vi "Configuration Tool Main.vi"() -> ()   [LabVIEW 2015, in "Configuration Tool.lvlib"]
doc: "This is the main VI for the configuration editor."
uses:
  Configuration Tool.lvlib
  Controls/StateCluster.ctl
  <vilib>/NI/Configuration Framework/Repository/NISE_CEF_Repository.lvclass
  <vilib>/NI/Configuration Framework/Node/NodeRef.ctl
  <vilib>/NI/Configuration Framework/Node/NISE_CEF_Node.lvclass
  <vilib>/NI/Configuration Framework/Node/StandardEvents.ctl
  <vilib>/NI/Configuration Framework/Node/UserEventRef.ctl
  <vilib>/NI/Configuration Framework/Controls/EventCluster.ctl
  <vilib>/NI/Configuration Framework/Node/NodeChangeEvent.ctl
  <vilib>/NI/Configuration Framework/Node/CacheState.ctl
  <vilib>/NI/Configuration Framework/Node/RefreshUIEvent.ctl
  <vilib>/NI/Configuration Framework/Node/StopEvent.ctl
  <vilib>/NI/Configuration Framework/glyph manager/glyph manager.ctl
  <vilib>/picture/picture.llb/imagedata.ctl
  Controls/AddMessage.ctl
  Controls/MoveMessage.ctl
  <vilib>/Utility/error.llb/DialogType.ctl
  Classes/CustomDeviceRepo/CustomDeviceRepo.lvclass
  <vilib>/Utility/sysdir.llb/System Directory Type.ctl
  <vilib>/NI/AMC/Read Termination Message.vi
  <vilib>/NI/AMC/Create Single Message.vi
  <vilib>/NI/AMC/Update Message Routing Info.vi
  subVI/Global Settings.vi
  <vilib>/NI/AMC/Globals.vi
  <vilib>/NI/AMC/Send Message.vi
  <vilib>/NI/AMC/AMC.lvlib
  <vilib>/NI/Configuration Framework/NISE_CEF_TreeControl.lvlib
  <vilib>/NI/Configuration Framework/glyph manager/glyph manager.lvlib
panel:
  in  "Target Project":string(combo)
  in  "VeriStand Version":enum16{"2013", "2014", "2015", "2016"}(ring)=enum."2015"
  in  "View":string(tree)
  in  "Exit":bool
  out "Status":string
  # "Custom Device XML Editor"
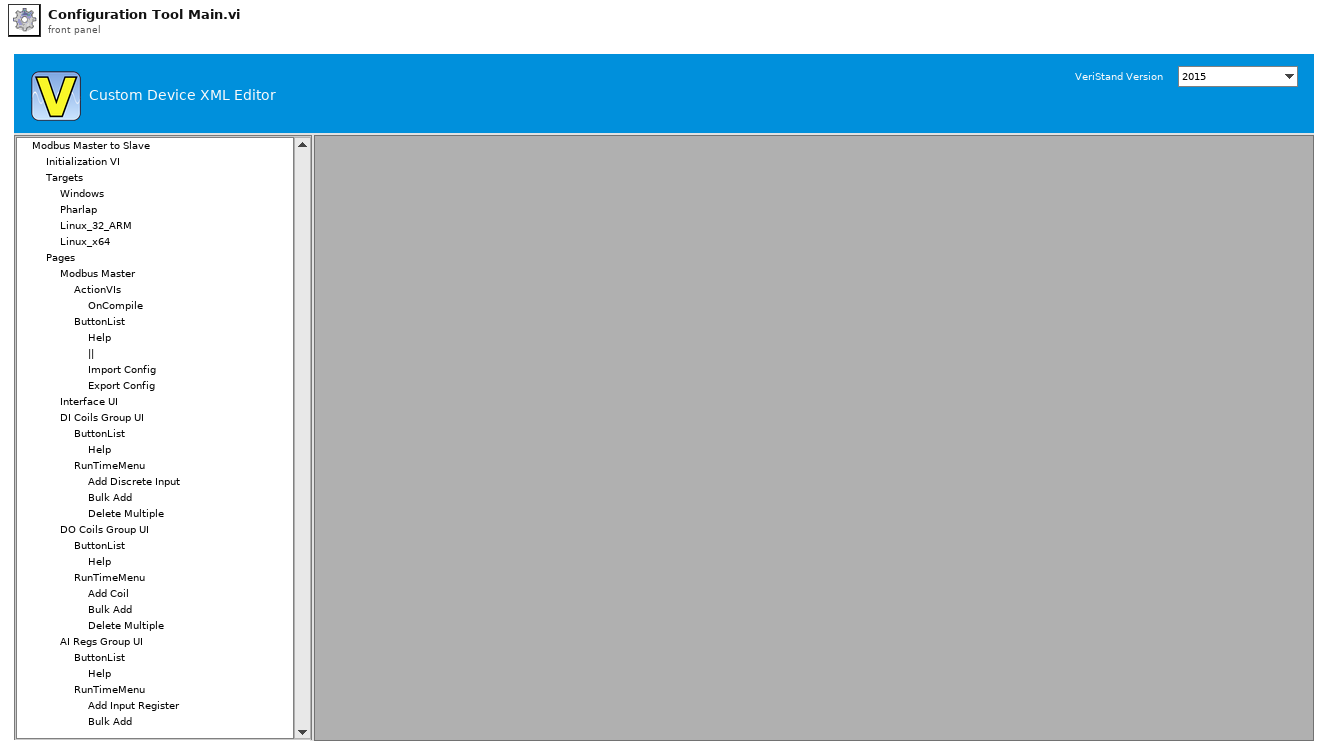
[diagram p1: front panel]
types:
  T1 = typedef "Configuration Tool.lvlib/StateCluster.ctl" = cluster{"repository":refnum<class "NISE_CEF_Repository.lvclass">, "root":T2, "unsaved changes":bool, "current path":path, "standard events":T3, "classes path":path, "glyph manager":T9}
  T2 = typedef "NISE_CEF_Node.lvclass/NodeRef.ctl" = refnum<data-value>
  T3 = typedef "NISE_CEF_Node.lvclass/StandardEvents.ctl" = cluster{"user event":T4, "node change":T5, "cache state":T6, "refresh UI":T7, "stop event":T8}
  T4 = typedef "NISE_CEF_Node.lvclass/UserEventRef.ctl" = refnum<user-event>
  T5 = typedef "NISE_CEF_Node.lvclass/NodeChangeEvent.ctl" = refnum<user-event>
  T6 = typedef "NISE_CEF_Node.lvclass/CacheState.ctl" = refnum<user-event>
  T7 = typedef "NISE_CEF_Node.lvclass/RefreshUIEvent.ctl" = refnum<user-event>
  T8 = typedef "NISE_CEF_Node.lvclass/StopEvent.ctl" = refnum<user-event>
  T9 = typedef "glyph manager.lvlib/glyph manager.ctl" = cluster{"search paths":path[], "glyph map":variant, "base glyphs":T10[], "desired overlays":string[]}
  T10 = typedef "imagedata.ctl" = cluster{"image type":i32, "image depth":i32, "image":u8[], "mask":u8[], "colors":u32[], "Rectangle":cluster{"left":i16, "top":i16, "right":i16, "bottom":i16}}
  T11 = cluster{"Names":string[], "Project refs":refnum<vi>[]}
  T12 = typedef "AMC.lvlib/Message Queue.ctl" = refnum<queue>
  T13 = typedef "Configuration Tool.lvlib/AddMessage.ctl" = cluster{"node type":string, "to add to":string}
  T14 = typedef "Configuration Tool.lvlib/MoveMessage.ctl" = cluster{"node ref":T2, "new parent":T2}
  T15 = typedef "Configuration Tool.lvlib/FilePaths.ctl" = cluster{"glyphs":path, "classes":path}
  T16 = typedef "DialogType.ctl" = u16
  T17 = typedef "System Directory Type.ctl" = i32
  T18 = typedef "NISE_CEF_Node.lvclass/Summary.ctl" = cluster{"ID":string, "parent ID":string, "node type":string, "text":string, "additional text":string, "glyph":string, "depth":i32, "glyph overlay":string}
  T19 = typedef "LVPoint32TypeDef.ctl" = cluster{"Horizontal":i32, "Vertical":i32}
  T20 = cluster{"data name":string, "drag data":variant}[]
  T21 = typedef "NISE_CEF_Node.lvclass/NodeMenuOptions.ctl" = cluster{"removable":bool, "movable":bool, "duplicate":bool}
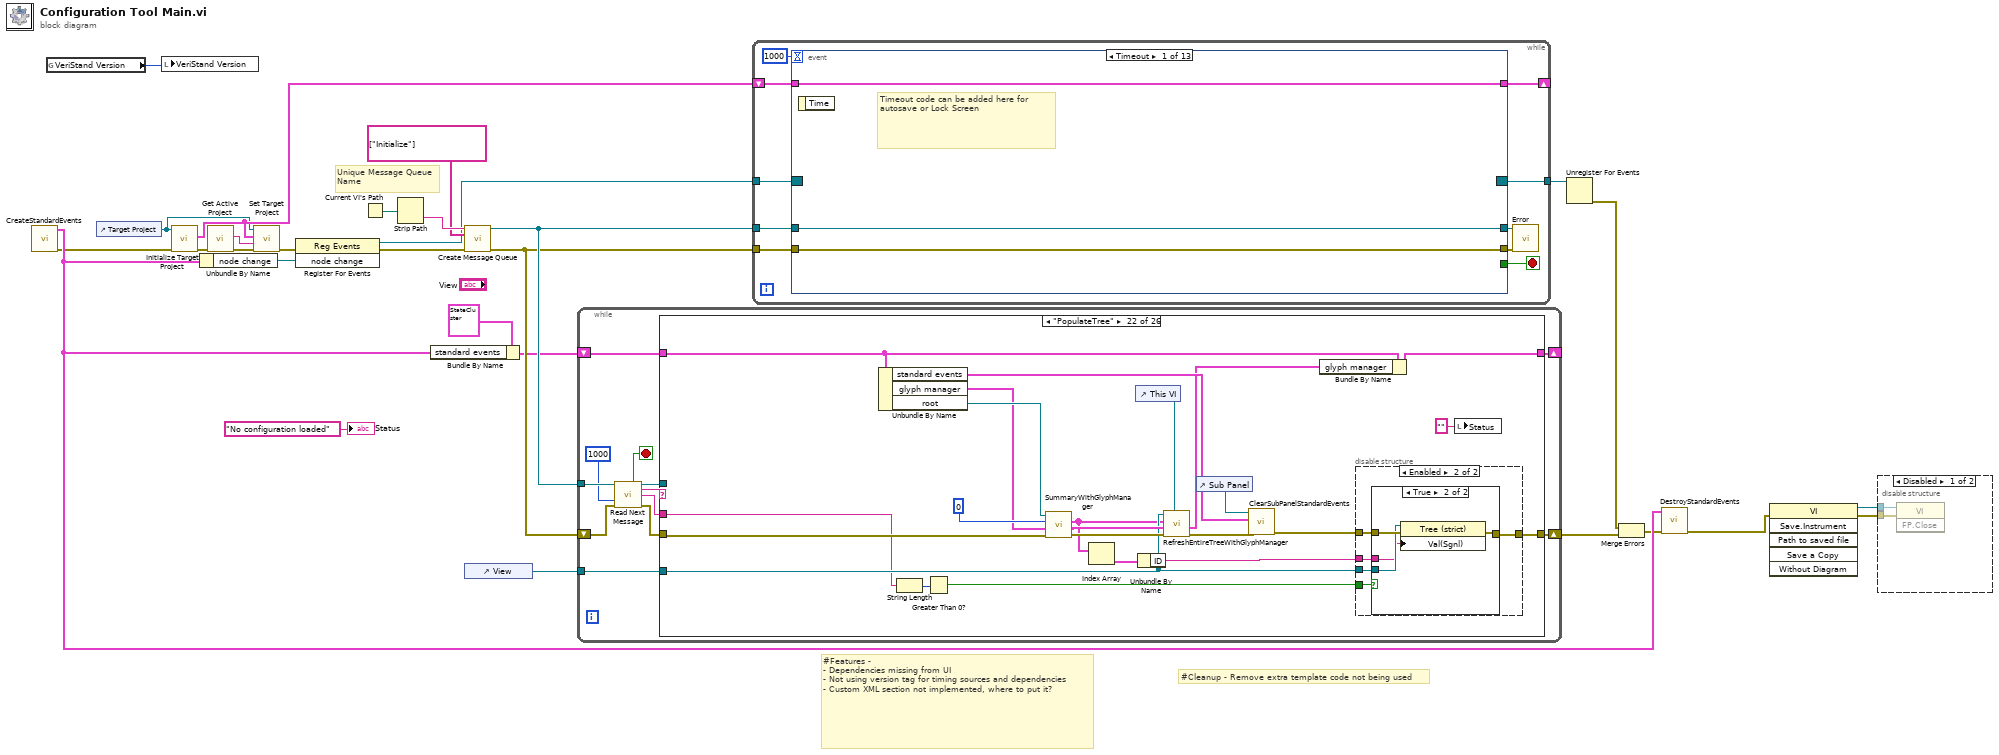
[diagram p0: block diagram]
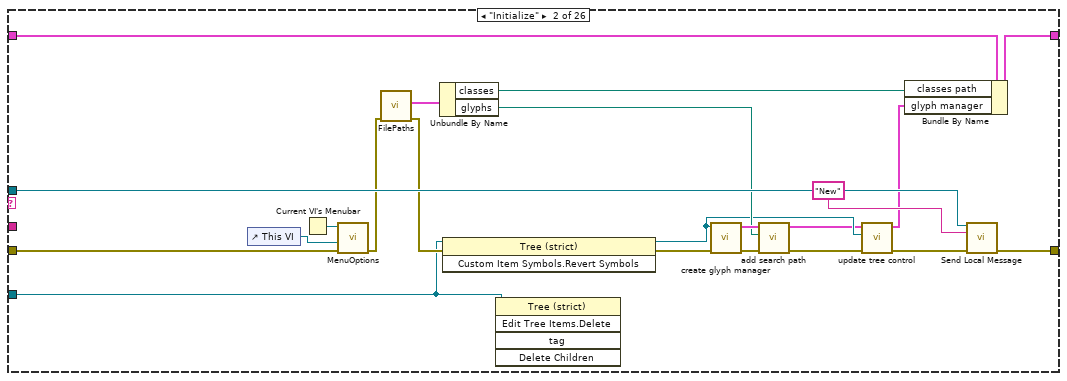
[diagram p4: hidden frame]
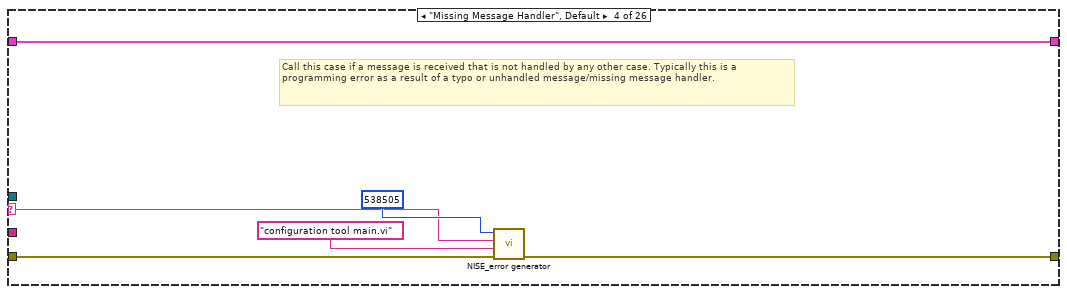
[diagram p6: hidden frame]
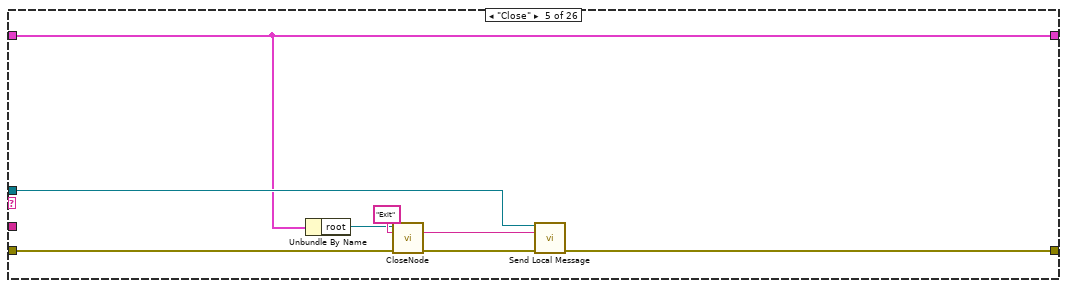
[diagram p7: hidden frame]
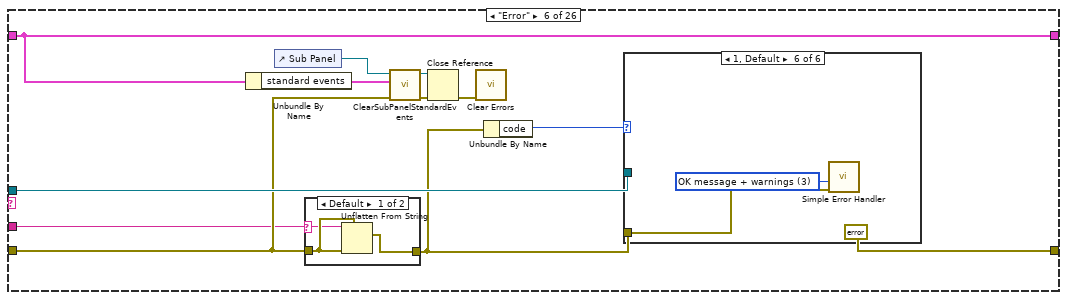
[diagram p8: hidden frame]
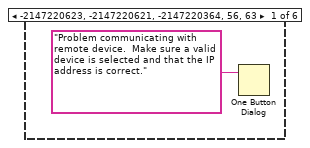
[diagram p10: hidden frame]
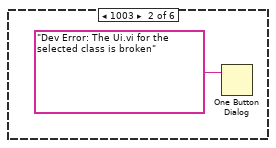
[diagram p11: hidden frame]
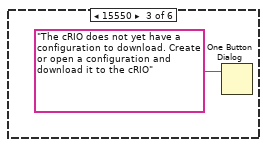
[diagram p12: hidden frame]
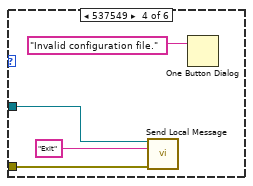
[diagram p13: hidden frame]
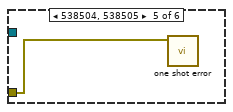
[diagram p14: hidden frame]
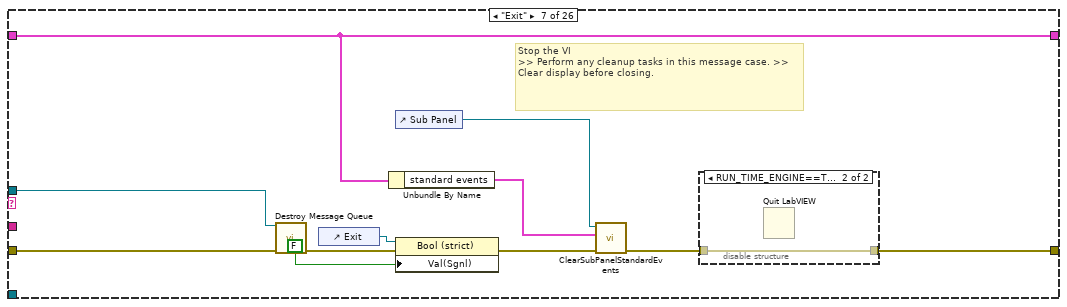
[diagram p15: hidden frame]
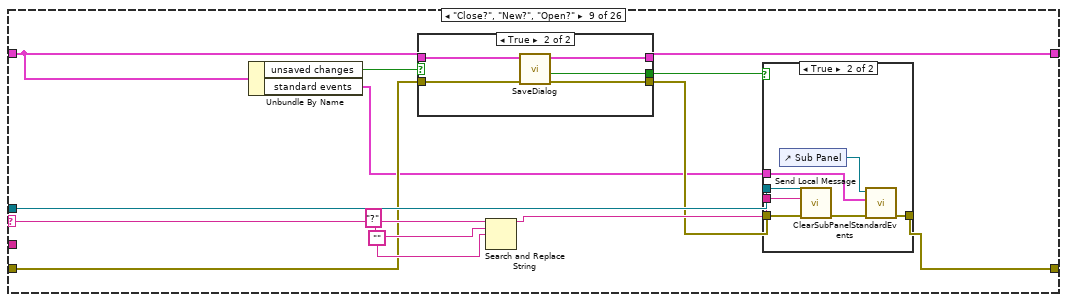
[diagram p18: hidden frame]
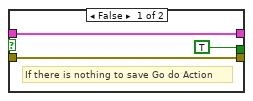
[diagram p19: hidden frame]
diagram:
  # "#Cleanup - Remove extra template code not being used"
  # "#Features - \n- Dependencies missing from UI\n- Not using version tag for timing sources and dependencies\n- Custom XML section not implemented, where to put it?"
  # "Unique Message Queue Name"
  n1 = call <vilib>:"CreateStandardEvents.vi"() -> ("error out"=w6:errorcluster, "standard events"=w18:T3)  [unwired: 10 in]
  n2 = global read "Global Settings.vi" "VeriStand Version"() -> (w12:enum16{"2013", "2014", "2015", "2016"})
  n3 = control-ref of="Target Project"() -> (w7:refnum<vi>)
  n4 = local write "VeriStand Version"(w12) -> ()
  n5 = call "Initialize Target Project.vi"("error in (no error)"=w6, "ComboBox in"=w7) -> ("error out"=w11:errorcluster, "Projects"=w9:T11)  [unwired: 8 in]
  n6 = Unbundle By Name(w18) -> ("node change"=w23:T5)
  n7 = call "Get Active Project.vi"("error in (no error)"=w11) -> ("error out"=w10:errorcluster, "Name"=w8:string)  [unwired: 7 in, 2 out]
  n8 = call "Set Target Project.vi"("error in (no error)"=w10, "Target Project"=w8, "Projects"=w9, "ComboBox Ref"=w7) -> ("error out"=w5:errorcluster)  [unwired: 7 in]
  n9 = register-events(error in=w5, w23) -> (reference out=w17:refnum<event-registration>, error out=w22:errorcluster)  [unwired: 1 in]
  n10 = Current VI's Path() -> (path=w27:path)
  n11 = Strip Path(path=w27) -> (name=w28:string)  [unwired: 1 out]
  n12 = Bundle By Name(cluster=T1 {"repository"=refnum, "root"=refnum, "unsaved changes"=FALSE, "current path"=path "", "standard events"={"user event"=refnum, "node change"=refnum, "cache state"=refnum, "refresh UI"=refnum, "stop event"=refnum}, "classes path"=path "", "glyph manager"={"search paths"=[], "glyph map"=variant, "base glyphs"=[], "desired overlays"=[]}}, "standard events"=w18) -> (w20:T1)
  n13 = call <vilib>:"Create Message Queue.vi"("message queue name"=w28, "initial message names"=string[] ["Initialize"], "error in"=w22) -> ("message queue out"=w25:T12, "error out"=w24:errorcluster)  [unwired: 11 in]
  n14 = control-ref of="View"() -> (w16:refnum<vi>)
  n15 = while "Message Processor" {
    shift-right: [w36] -> w19
    shift-left: w24 -> [w35]
    tunnel: w25 -> [w34]
    shift-right: [w32] -> _
    shift-left: w20 -> [w31]
    tunnel: w16 -> [w29]
    stop <- w40 stop-if-true
    n16 = call <vilib>:"Read Next Message.vi"("message queue in"=w34, "timeout (1 ms)"=1000, "error in"=w35) -> ("exit process?"=w40:bool, "message queue out"=w30:T12, "message name"=w39:string, "message value"=w38:string, "error out"=w37:errorcluster)  [unwired: 5 in, 3 out]
    n17 = case shown="\"PopulateTree\"" w39 {
      selector: w39 -> [_ _ _ w68 _ _ _ _ w129 _ _ _ _ _ _ _ _ _ w385 _ _ _ _ _ _ _]
      tunnel: w38 -> [_ _ _ _ _ w81 _ _ _ _ _ _ _ _ w294 _ w346 w363 w383 w435 w459 w471 _ w520 w540 w547]
      tunnel: w37 -> [w42 w64 w66 w71 w74 w84 w116 w120 w122 w160 w180 w220 w264 w286 w301 w314 w339 w362 w388 w437 w458 w488 w510 w519 w538 w548]
      tunnel: [w42 w60 w66 w69 w78 errorcluster {"status"=FALSE, "code"=0, "source"=""} ("error out") w108 w120 w133 w166 w176 w225 w261 w288 w298 w314 w318 w366 w391 w439 w455 w475 w506 w516 w533 w546] -> w36
      tunnel: [w41 w56 w65 w72 w76 w88 w107 w119 w124 w164 w181 w228 w267 w287 w295 w313 w334 w359 w392 w438 w460 w481 w509 w514 w541 w543] -> w32
      tunnel: w31 -> [w41 w57 w65 w72 w76 w88 w107 w119 w125 w162 w182 w229 w266 w285 w296 w313 w337 w360 w392 w430 w460 w490 w509 w514 w541 w549]
      tunnel: w30 -> [_ w59 _ _ w77 w91 w115 _ w132 w165 w178 w227 _ _ w297 _ w315 _ w386 _ _ _ _ w515 w532 w545]
      tunnel: w29 -> [_ w43 _ _ _ _ _ _ _ _ _ _ _ _ _ _ w335 w355 w380 w432 w453 w477 _ _ _ _]
      frame "------------Generic Operations------------" {
        # "Dummy case to add a seperation in the Case Structure menu"
      }
      frame "Initialize" {
        n18 = control-ref of="This VI"() -> (w63:refnum<vi>)
        n19 = Current VI's Menubar() -> (w62:refnum<k9>)
        n20 = call "MenuOptions.vi"("error in"=w64, "VI ref"=w63, "menu ref in"=w62) -> ("error out"=w55:errorcluster)  [unwired: 7 in, 1 out]
        n21 = call "FilePaths.vi"("error in"=w55) -> ("error out"=w48:errorcluster, "paths"=w58:T15)  [unwired: 9 in]
        n22 = Unbundle By Name(w58) -> ("classes"=w54:path, "glyphs"=w50:path)
        n23 = invoke class="Tree (strict)" method="Custom Item Symbols.Revert Symbols"(reference=w43, error in=w48) -> (reference out=w46:refnum<vi>, error out=w47:errorcluster)  [unwired: 1 in, 1 out]
        n24 = invoke class="Tree (strict)" method="Edit Tree Items.Delete"(reference=w43) -> ()  [unwired: 4 in, 5 out]
        n25 = call <vilib>:"create glyph manager.vi"("error in"=w47, "tree ref (for default symbols)"=w46) -> ("error out"=w53:errorcluster, "glyph manager"=w52:T9)  [unwired: 8 in]
        n26 = call <vilib>:"add search path.vi"("error in"=w53, "search path"=w50, "glyph manager in"=w52) -> ("error out"=w45:errorcluster, "glyph manager out"=w44:T9)  [unwired: 7 in]
        n27 = call <vilib>:"update tree control.vi"("error in"=w45, "tree reference"=w46, "glyph manager in"=w44) -> ("error out"=w51:errorcluster, "glyph manager out"=w49:T9)  [unwired: 7 in]
        n28 = Bundle By Name(cluster=w57, "classes path"=w54, "glyph manager"=w49) -> (w56:T1)
        n29 = call <vilib>:"Send Local Message.vi"("message queue in"=w59, "message name"="New" ("Message Name"), "error in"=w51) -> ("error out"=w60:errorcluster)  [unwired: 10 in, 2 out]
      }
      frame "", "Idle" {
      }
      frame "Missing Message Handler", Default {
        # "Call this case if a message is received that is not handled by any other case. Typically this is a programming error as a result of a typo or unhandled message/missing message handler."
        n30 = call <vilib>:"NISE_error generator.vi"("error in"=w71, "source"="configuration tool main.vi", "append error message"=w68, "error code (0)"=538505) -> ("error out"=w69:errorcluster)  [unwired: 5 in]
      }
      frame "Close" {
        n31 = Unbundle By Name(w76) -> ("root"=w75:T2)
        n32 = call <vilib>:"CloseNode.vi"("error in"=w74, "node ref"=w75) -> ("error out"=w73:errorcluster)  [unwired: 9 in]
        n33 = call <vilib>:"Send Local Message.vi"("message queue in"=w77, "message name"="Exit", "error in"=w73) -> ("error out"=w78:errorcluster)  [unwired: 10 in, 2 out]
      }
      frame "Error" {
        n34 = Unbundle By Name(w88) -> ("standard events"=w80:T3)
        n35 = control-ref of="Sub Panel"() -> (w87:refnum<vi>)
        n36 = case shown="Default" w81 {
          selector: w81 -> [w93 _]
          tunnel: w84 -> [w94 w95]
          tunnel: [w92 w95] -> w83
          frame Default {
            n37 = Unflatten From String(type=w94, binary string=w93, error in (no error)=w94) -> (value=w92:errorcluster)  [unwired: 2 in, 2 out]
          }
          frame "" {
          }
        }
        n38 = call <vilib>:"ClearSubPanelStandardEvents.vi"("error in"=w84, "standard events"=w80, "sub panel ref in"=w87) -> ("error out"=w86:errorcluster, "sub panel ref out"=w85:refnum<vi>)  [unwired: 7 in]
        n39 = Close Reference(reference=w85, error in (no error)=w86) -> (error out=w82:errorcluster)
        n40 = call <vilib>:"Clear Errors.vi"("error in (no error)"=w82) -> ()  [unwired: 5 in, 2 out]
        n41 = Unbundle By Name(w83) -> ("code"=w89:i32)
        n42 = case shown="1, Default" w89 {
          tunnel: w91 -> [_ _ _ w101 _ _]
          tunnel: w83 -> [_ _ _ w100 w103 w105]
          frame -2147220623, -2147220621, -2147220364, 56, 63 {
            n43 = One Button Dialog(message="Problem communicating with remote device.  Make sure a valid device is selected and that the IP address is correct.") -> ()  [unwired: 1 in, 1 out]
          }
          frame 1003 {
            n44 = One Button Dialog(message="Dev Error: The Ui.vi for the selected class is broken") -> ()  [unwired: 1 in, 1 out]
          }
          frame 15550 {
            n45 = One Button Dialog(message="The cRIO does not yet have a configuration to download. Create or open a configuration and download it to the cRIO") -> ()  [unwired: 1 in, 1 out]
          }
          frame 537549 {
            n46 = call <vilib>:"Send Local Message.vi"("message queue in"=w101, "message name"="Exit", "error in"=w100) -> ()  [unwired: 10 in, 3 out]
            n47 = One Button Dialog(message="Invalid configuration file.") -> ()  [unwired: 1 in, 1 out]
          }
          frame 538504, 538505 {
            n48 = call <vilib>:"one shot error.vi"("error in"=w103) -> ()  [unwired: 11 in]
          }
          frame 1, Default {
            w104 = T16 3 items=["no dialog", "OK message", "continue or stop message", "OK message + warnings", "continue/stop + warnings"] ("type of dialog (OK msg:1)")
            n49 = call <vilib>:"Simple Error Handler.vi"("type of dialog (OK msg:1)"=w104, "error in (no error)"=w105) -> ()  [unwired: 8 out]
          }
        }
      }
      frame "Exit" {
        # "Stop the VI                                                                             >> Perform any cleanup tasks in this message case. >> Clear display before closing."
        n50 = call <vilib>:"Destroy Message Queue.vi"("message queue in"=w115, "error in"=w116) -> ("error out"=w112:errorcluster)  [unwired: 11 in, 2 out]
        n51 = control-ref of="Exit"() -> (w114:refnum<vi>)
        n52 = Unbundle By Name(w107) -> ("standard events"=w106:T3)
        n53 = control-ref of="Sub Panel"() -> (w111:refnum<vi>)
        n54 = property class="Bool (strict)"(reference=w114, error in=w112, "Val(Sgnl)"=FALSE ("Exit")) -> (error out=w110:errorcluster)  [unwired: 1 out]
        n55 = call <vilib>:"ClearSubPanelStandardEvents.vi"("error in"=w110, "standard events"=w106, "sub panel ref in"=w111) -> ("error out"=w109:errorcluster)  [unwired: 7 in, 1 out]
        n56 = disable-structure shown="RUN_TIME_ENGINE==True" {
          disable-tunnel: [w117 w118] -> w108
          disable-tunnel: w109 -> [w117 w118]
          frame condition #0 (active) {
          }
          frame condition #1 {
            n57 = Quit LabVIEW() -> ()  [unwired: 1 in]
          }
        }
      }
      frame "------------Menu Operations--------------" {
        # "Dummy case to add a seperation in the Case Structure menu"
      }
      frame "Close?", "New?", "Open?" {
        n58 = Unbundle By Name(w125) -> ("unsaved changes"=w127:bool, "standard events"=w121:T3)
        n59 = case shown="True" w127 {
          tunnel: [TRUE ("SaveFlag") w141] -> w126
          tunnel: w125 -> [w135 w140]
          tunnel: [w135 w139] -> w124
          tunnel: w122 -> [w134 w138]
          tunnel: [w134 w137] -> w123
          frame False {
            # "If there is nothing to save Go do Action"
          }
          frame True {
            n60 = call "SaveDialog.vi"("error in"=w138, "state in"=w140) -> ("error out"=w137:errorcluster, "new"=w141:bool, "state out"=w139:T1)  [unwired: 7 in]
          }
        }
        n61 = Search and Replace String(input string=w129, search string="?", replace string="") -> (result string=w128:string)  [unwired: 5 in, 3 out]
        n62 = case shown="True" w126 {
          tunnel: w123 -> [w142 w149]
          tunnel: [w142 w145] -> w133
          tunnel: w132 -> [_ w148]
          tunnel: w128 -> [_ w147]
          tunnel: w121 -> [_ w143]
          frame False {
          }
          frame True {
            n63 = control-ref of="Sub Panel"() -> (w144:refnum<vi>)
            n64 = call <vilib>:"Send Local Message.vi"("message queue in"=w148, "message name"=w147, "error in"=w149) -> ("error out"=w146:errorcluster)  [unwired: 10 in, 2 out]
            n65 = call <vilib>:"ClearSubPanelStandardEvents.vi"("error in"=w146, "standard events"=w143, "sub panel ref in"=w144) -> ("error out"=w145:errorcluster)  [unwired: 7 in, 1 out]
          }
        }
      }
      frame "New" {
        # "#Change - Won't allow creating so changing unsaved constant to F"
        n66 = Unbundle By Name(w162) -> ("classes path"=w161:path)
        n67 = Current VI's Menubar() -> (w156:refnum<k9>)
        n68 = call-dynamic "Initialize.vi"("error in"=w160, "path"=w161, "repository in"=refnum<class "CustomDeviceRepo.lvclass"> refnum ("CustomDeviceRepo.lvclass")) -> ("error out"=w159:errorcluster, "repository out"=w158:refnum<class "CustomDeviceRepo.lvclass">)  [unwired: 7 in]
        n69 = call-dynamic "GenerateMenu.vi"("error in"=w159, "menu ref in"=w156, "NISE_CEF_Repository in"=w158) -> ("error out"=w155:errorcluster, "NISE_CEF_Repository out"=w157:refnum<class "CustomDeviceRepo.lvclass">)  [unwired: 6 in, 1 out]
        n70 = call "Get Active Project.vi"() -> ("No Active Project?"=w153:bool)  [unwired: 8 in, 3 out]
        n71 = Bundle By Name(cluster=w162, "unsaved changes"=FALSE ("SaveFlag"), "repository"=w157) -> (w164:T1)
        n72 = Select(t="Idle", s=w153, f="Open Active") -> (s? t:f=w150:string)
        n73 = call <vilib>:"Send Local Message.vi"("message queue in"=w165, "message name"=w150, "error in"=w155) -> ("error out"=w166:errorcluster)  [unwired: 10 in, 2 out]
      }
      frame "Open" {
        w175 = T17 6 items=["User Home"=0, "User Desktop"=1, "User Documents"=2, "User Application Data"=3, "User Preferences"=4, "User Temporary"=5, "Public Documents"=6, "Public Application Data"=7, "Public Preferences"=8, "Public Cache"=13, "System Core Libraries"=9, "System Installed Libraries"=10, "Application Files"=11, "Boot Volume Root"=12] ("system directory type")
        n74 = global read "Global Settings.vi" "VeriStand Version"() -> (w168:enum16{"2013", "2014", "2015", "2016"})
        n75 = Format Into String(w168) -> (resulting string=w167:string)  [unwired: 3 in, 1 out]
        n76 = Search and Replace String(input string="National Instruments\\NI VeriStand XXXX\\Custom Devices", search string="XXXX", replace string=w167) -> (result string=w171:string)  [unwired: 5 in, 3 out]
        n77 = call <vilib>:"Get System Directory.vi"("system directory type"=w175) -> ("system directory"=w172:path)  [unwired: 10 in]
        n78 = Build Path(base path=w172, name or relative path=w171) -> (appended path=w170:path)
        n79 = in-place {
          in-place-border: w180 -> [w188]
          in-place-border: [w187] -> w177
          in-place-border: w170 -> [w183]
          n80 = in-place-cluster #1(w182) -> ("current path"=w185:path, "repository"=w196:refnum<class "NISE_CEF_Repository.lvclass">, "root"=w192:T2)  [unwired: 1 out]
          n81 = call "FileDialog.vi"("error in"=w188, "start path"=w183) -> ("error out"=w189:errorcluster, "cancelled"=w190:bool, "selected path"=w186:path)  [unwired: 7 in]
          n82 = Compound Arithmetic op=OR(invert w190) -> (w191:bool)
          n83 = case shown="True" w191 {
            tunnel: w196 -> [w197 w209]
            tunnel: [w197 w207] -> w194
            tunnel: [w198 w205] -> w187
            tunnel: [w199 w204] -> w193
            tunnel: w186 -> [_ w202]
            tunnel: w189 -> [w198 w201]
            tunnel: w192 -> [w199 w200]
            frame False {
            }
            frame True {
              n84 = call-dynamic "Open.vi"("error in"=w201, "file path"=w202, "repository in"=w209) -> ("error out"=w206:errorcluster, "invalid?"=w203:bool, "repository out"=w208:refnum<class "NISE_CEF_Repository.lvclass">)  [unwired: 6 in]
              n85 = case shown="False" w203 {
                tunnel: w208 -> [w214 w217]
                tunnel: [w213 w217] -> w207
                tunnel: w206 -> [w212 w216]
                tunnel: [w211 w216] -> w205
                tunnel: [w210 w215] -> w204
                tunnel: w200 -> [_ w215]
                frame False {
                  n86 = call-dynamic "WriteTree.vi"("error in"=w212, "repository in"=w214) -> ("error out"=w211:errorcluster, "root"=w210:T2, "repository out"=w213:refnum<class "NISE_CEF_Repository.lvclass">)  [unwired: 7 in]
                }
                frame True {
                }
              }
            }
          }
          n87 = Select(t=w185, s=w187, f=w186) -> (s? t:f=w184:path)
          n88 = in-place-cluster #1("current path"=w184, "unsaved changes"=FALSE ("SaveFlag"), "repository"=w194, "root"=w193) -> (w181:T1)
        }
        n89 = call <vilib>:"Send Local Message.vi"("message queue in"=w178, "message name"="PopulateTree", "message value"="Zero", "error in"=w177) -> ("error out"=w176:errorcluster)  [unwired: 9 in, 2 out]
      }
      frame "Open Active" {
        n90 = global read "Global Settings.vi" "Target Project Ref"() -> (w223:refnum<vi>)
        n91 = call "Search Project for XML Files.vi"("error in (no error)"=w220, "project reference"=w223) -> ("error out"=w219:errorcluster, "xml files found"=w222:path[])  [unwired: 8 in]
        n92 = Empty Array?(array=w222) -> (empty?=w221:bool)
        n93 = case shown="True" w221 {
          tunnel: w229 -> [w236 w260]
          tunnel: [w235 w260] -> w228
          tunnel: w219 -> [w234 w259]
          tunnel: [w233 w259] -> w226
          tunnel: w222 -> [w231 _]
          tunnel: ["PopulateTree" "Idle"] -> w218
          frame False {
            n94 = Index Array(array=w231) -> (element=w232:path)  [unwired: 1 in]
            n95 = in-place {
              in-place-border: w234 -> [w244]
              in-place-border: [w243] -> w233
              in-place-border: w232 -> [w237]
              n96 = in-place-cluster #2(w236) -> ("current path"=w242:path, "repository"=w249:refnum<class "NISE_CEF_Repository.lvclass">, "root"=w245:T2)  [unwired: 1 out]
              n97 = call-dynamic "Open.vi"("error in"=w244, "file path"=w237, "repository in"=w249) -> ("error out"=w239:errorcluster, "invalid?"=w238:bool, "repository out"=w240:refnum<class "NISE_CEF_Repository.lvclass">)  [unwired: 6 in]
              n98 = case shown="False" w238 {
                tunnel: w240 -> [w254 w257]
                tunnel: [w253 w257] -> w247
                tunnel: w239 -> [w252 w256]
                tunnel: [w251 w256] -> w243
                tunnel: [w250 w255] -> w246
                tunnel: w245 -> [_ w255]
                frame False {
                  n99 = call-dynamic "WriteTree.vi"("error in"=w252, "repository in"=w254) -> ("error out"=w251:errorcluster, "root"=w250:T2, "repository out"=w253:refnum<class "NISE_CEF_Repository.lvclass">)  [unwired: 7 in]
                }
                frame True {
                }
              }
              n100 = Select(t=w242, s=w243, f=w237) -> (s? t:f=w241:path)
              n101 = in-place-cluster #2("current path"=w241, "unsaved changes"=FALSE ("SaveFlag"), "repository"=w247, "root"=w246) -> (w235:T1)
            }
          }
          frame True {
          }
        }
        n102 = call <vilib>:"Send Local Message.vi"("message queue in"=w227, "message name"=w218, "message value"="Zero", "error in"=w226) -> ("error out"=w225:errorcluster)  [unwired: 9 in, 2 out]
      }
      frame "Save" {
        n103 = in-place {
          in-place-border: w264 -> [w271]
          in-place-border: [w270] -> w263
          in-place-border: [w268] -> w262
          n104 = in-place-cluster #3(w266) -> ("current path"=w269:path, "root"=w272:T2, "repository"=w274:refnum<class "NISE_CEF_Repository.lvclass">)
          n105 = Empty String/Path?(string/path=w269) -> (empty?=w268:bool)
          n106 = call-dynamic "ReadTree.vi"("error in"=w271, "root"=w272, "repository in"=w274) -> ("error out"=w270:errorcluster, "repository out"=w273:refnum<class "NISE_CEF_Repository.lvclass">)  [unwired: 7 in]
          n107 = in-place-cluster #3("current path"=w269, "root"=w272, "repository"=w273) -> (w265:T1)
        }
        n108 = case shown="False" w262 {
          tunnel: w265 -> [w278 w280]
          tunnel: [w277 w279] -> w267
          tunnel: [w276 w281] -> w261
          tunnel: w263 -> [w275 w282]
          frame False {
            n109 = call "Save.vi"("error in"=w275, "state in"=w278) -> ("error out"=w276:errorcluster, "state out"=w277:T1)  [unwired: 8 in]
          }
          frame True {
            # "Empty path use Dialog"
            n110 = call "SaveAs.vi"("error in"=w282, "state in"=w280) -> ("error out"=w281:errorcluster, "state out"=w279:T1)  [unwired: 7 in, 1 out]
          }
        }
      }
      frame "SaveAs" {
        n111 = in-place {
          in-place-border: w286 -> [w290]
          in-place-border: [w289] -> w284
          n112 = in-place-cluster #4(w285) -> ("root"=w291:T2, "repository"=w293:refnum<class "NISE_CEF_Repository.lvclass">)
          n113 = call-dynamic "ReadTree.vi"("error in"=w290, "root"=w291, "repository in"=w293) -> ("error out"=w289:errorcluster, "repository out"=w292:refnum<class "NISE_CEF_Repository.lvclass">)  [unwired: 7 in]
          n114 = in-place-cluster #4("root"=w291, "repository"=w292) -> (w283:T1)
        }
        n115 = call "SaveAs.vi"("error in"=w284, "state in"=w283) -> ("error out"=w288:errorcluster, "state out"=w287:T1)  [unwired: 7 in, 1 out]
      }
      frame "Custom View" {
        n116 = in-place {
          in-place-border: w301 -> [w312]
          in-place-border: [w311] -> w299
          in-place-border: w294 -> [w302]
          n117 = in-place-cluster #5(w296) -> ("repository"=w306:refnum<class "NISE_CEF_Repository.lvclass">, "root"=w305:T2)
          n118 = call-dynamic "ReadTree.vi"("error in"=w312, "root"=w305, "repository in"=w306) -> ("error out"=w309:errorcluster, "repository out"=w308:refnum<class "NISE_CEF_Repository.lvclass">)  [unwired: 7 in]
          n119 = call-dynamic "CustomView.vi"("error in"=w309, "view name"=w302, "repository in"=w308) -> ("error out"=w310:errorcluster, "repository out"=w307:refnum<class "NISE_CEF_Repository.lvclass">)  [unwired: 7 in]
          n120 = call-dynamic "WriteTree.vi"("error in"=w310, "repository in"=w307) -> ("error out"=w311:errorcluster, "root"=w303:T2, "repository out"=w304:refnum<class "NISE_CEF_Repository.lvclass">)  [unwired: 7 in]
          n121 = in-place-cluster #5("repository"=w304, "root"=w303) -> (w295:T1)
        }
        n122 = call <vilib>:"Send Local Message.vi"("message queue in"=w297, "message name"="PopulateTree", "error in"=w299) -> ("error out"=w298:errorcluster)  [unwired: 10 in, 2 out]
      }
      frame "-------TreeControl Operations-----------" {
        # "Dummy case to add a seperation in the Case Structure menu"
      }
      frame "AddNode" {
        # "#Change - Added ability for added nodes\nto then add children"
        # "#Change - Had to make own copy\nof add node since CEF framework\ndoesn't let you pass params to init"
        # "#Change - Look for potential\ndashes for menu items with\nparameterized options"
        n123 = Unflatten From String(type=T13 {"node type"="", "to add to"=""} ("input cluster"), binary string=w346) -> (value=w344:T13)  [unwired: 3 in, 2 out]
        n124 = Unbundle By Name(w344) -> ("to add to"=w342:string, "node type"=w324:string)
        n125 = Match Pattern(string=w324, regular expression="\\-") -> (before substring=w323:string, after substring=w322:string)  [unwired: 1 in, 2 out]
        n126 = in-place {
          in-place-border: w339 -> [w352]
          in-place-border: [w351] -> w338
          in-place-border: w323 -> [w350]
          in-place-border: [w349] -> w336
          n127 = in-place-cluster #6(w337) -> ("repository"=w354:refnum<class "NISE_CEF_Repository.lvclass">)
          n128 = call-dynamic "GetClassPath.vi"("error in"=w352, "class name"=w350, "Repository in"=w354) -> ("error out"=w351:errorcluster, "class path"=w349:path, "Repository out"=w353:refnum<class "NISE_CEF_Repository.lvclass">)  [unwired: 6 in]
          n129 = in-place-cluster #6("repository"=w353) -> (w331:T1)
        }
        n130 = Unbundle By Name(w331) -> ("glyph manager"=w330:T9)
        n131 = call <vilib>:"Get LV Class Default Value.vi"("error in (no error)"=w338, "class path"=w336) -> ("error out"=w347:errorcluster, "object"=w348:refnum<class>)  [unwired: 8 in]
        n132 = To More Specific Class(target class=refnum<class "NISE_CEF_Node.lvclass"> refnum ("Node.lvclass"), reference=w348, error in=w347) -> (specific class reference=w332:refnum<class "NISE_CEF_Node.lvclass">, error out=w333:errorcluster)
        n133 = call-dynamic "AddGlyphtoGManager.vi"("error in"=w333, "glyph manager"=w330, "NISE_CEF_Node in"=w332) -> ("error out"=w328:errorcluster, "glyph manager out"=w329:T9, "NISE_CEF_Node out"=w327:refnum<class "NISE_CEF_Node.lvclass">)  [unwired: 6 in]
        n134 = Match Pattern(string=w322, regular expression="\\-") -> (before substring=w320:string, after substring=w317:string)  [unwired: 1 in, 2 out]
        n135 = call "Modified Framework AddNode.vi"("parameters"=w320, "error in"=w328, "node in"=w327, "parent node ID"=w342) -> ("error out"=w341:errorcluster, "summary"=w340:T18[], "ID of Added Node"=w316:string)  [unwired: 5 in]
        n136 = call <vilib>:"PopulateTreeSumaryWithGlyphManager.vi"("error in"=w341, "glyph manager"=w329, "summary"=w340, "tree ref in"=w335) -> ("error out"=w319:errorcluster, "glyph manager out"=w326:T9)  [unwired: 6 in]
        n137 = Bundle By Name(cluster=w331, "glyph manager"=w326) -> (w334:T1)
        n138 = call "Send Message to Create Child Object.vi"("Error In"=w319, "ID of Node to Add To"=w316, "node type"=w317, "Queue in"=w315) -> ("Error Out"=w318:errorcluster)  [unwired: 6 in, 1 out]
      }
      frame "Duplicate" {
        n139 = call <vilib>:"IDtoNode.vi"("error in"=w362, "ID"=w363) -> ("error out"=w364:errorcluster, "invalid Id"=w361:bool, "node ref"=w365:T2)  [unwired: 7 in]
        n140 = Unbundle By Name(w360) -> ("glyph manager"=w357:T9)
        n141 = case shown="False" w361 {
          tunnel: [w377 w379] -> w366
          tunnel: w365 -> [w376 _]
          tunnel: w364 -> [w373 w379]
          tunnel: w357 -> [w369 w378]
          tunnel: [w368 w378] -> w356
          tunnel: w355 -> [w367 _]
          frame False {
            n142 = call <vilib>:"DuplicateNode.vi"("same parent?"=TRUE ("s"), "error in"=w373, "node ref in"=w376) -> ("error out"=w374:errorcluster, "new node ref"=w375:T2)  [unwired: 7 in]
            n143 = call <vilib>:"Summary.vi"("error in"=w374, "node self ref"=w375) -> ("error out"=w371:errorcluster, "summary"=w370:T18[])  [unwired: 8 in]
            n144 = call <vilib>:"PopulateTreeSumaryWithGlyphManager.vi"("error in"=w371, "glyph manager"=w369, "summary"=w370, "tree ref in"=w367) -> ("error out"=w377:errorcluster, "glyph manager out"=w368:T9)  [unwired: 6 in]
          }
          frame True {
          }
        }
        n145 = Bundle By Name(cluster=w360, "unsaved changes"=TRUE, "glyph manager"=w356) -> (w359:T1)
      }
      frame "CustomMenuAction" {
        n146 = Match Pattern(string=w383, regular expression=":") -> (before substring=w382:string, after substring=w381:string)  [unwired: 1 in, 2 out]
        n147 = call <vilib>:"IDtoNode.vi"("error in"=w388, "ID"=w381) -> ("error out"=w389:errorcluster, "invalid Id"=w387:bool, "node ref"=w390:T2)  [unwired: 7 in]
        n148 = case shown="False" w387 {
          tunnel: [w398 w428] -> w391
          tunnel: w390 -> [w395 _]
          tunnel: w389 -> [w401 w428]
          tunnel: w386 -> [w402 _]
          tunnel: w385 -> [_ _]
          tunnel: w382 -> [w399 _]
          tunnel: w380 -> [w396 _]
          frame False {
            n149 = in-place {
              in-place-border: w402 -> [w426]
              in-place-border: w401 -> [w424]
              in-place-border: [w423] -> w397
              in-place-border: [w422] -> w400
              in-place-border: w399 -> [w421]
              in-place-border: w396 -> [w420]
              in-place-border: [w419] -> w394
              n150 = in-place-dvr #7(w395) -> (w427:refnum<class "NISE_CEF_Node.lvclass">)  [unwired: 1 out]
              n151 = call-dynamic "MenuHandler.vi"("tree control"=w420, "main message queue"=w426, "error in"=w424, "menu string"=w421, "NISE_CEF_Node in"=w427) -> ("error out"=w423:errorcluster, "refresh tree?"=w419:bool, "Unhandled"=w422:bool, "NISE_CEF_Node out"=w425:refnum<class "NISE_CEF_Node.lvclass">)  [unwired: 3 in]
              n152 = in-place-dvr #7(w425) -> (w393:T2)  [unwired: 1 out]
            }
            n153 = case shown="True" w400 {
              tunnel: w399 -> [_ w414]
              tunnel: [w406 w415] -> w398
              tunnel: w397 -> [w404 w416]
              tunnel: w394 -> [w403 _]
              tunnel: w393 -> [w405 _]
              frame False {
                n154 = case shown="True" w403 {
                  tunnel: [w407 w410] -> w406
                  tunnel: w405 -> [_ w409]
                  tunnel: w404 -> [w407 w408]
                  frame False {
                  }
                  frame True {
                    n155 = call <vilib>:"NodetoID.vi"("error in"=w408, "node ref"=w409) -> ("error out"=w412:errorcluster, "ID"=w413:string)  [unwired: 8 in]
                    n156 = call <vilib>:"Send Local Message.vi"("message name"="NodeDataChange", "message value"=w413, "error in"=w412) -> ("error out"=w410:errorcluster)  [unwired: 10 in, 2 out]
                  }
                }
              }
              frame True {
                n157 = call <vilib>:"NISE_error generator.vi"("error in"=w416, "source"="configuration tool main.vi", "append error message"=w414, "error code (0)"=538506) -> ("error out"=w415:errorcluster)  [unwired: 5 in]
              }
            }
          }
          frame True {
          }
        }
      }
      frame "RefreshNode" {
        # "Refreshes the node in the Tree, Sets the save flag to true. This case can be called from the UIs of the nodes"
        n158 = Unbundle By Name(w430) -> ("glyph manager"=w429:T9)
        n159 = call <vilib>:"IDtoNode.vi"("error in"=w437, "ID"=w435) -> ("error out"=w436:errorcluster, "invalid Id"=w433:bool, "node ref"=w434:T2)  [unwired: 7 in]
        n160 = case shown="False" w433 {
          tunnel: [w449 w452] -> w439
          tunnel: w436 -> [w445 w452]
          tunnel: w434 -> [w444 _]
          tunnel: w432 -> [w443 _]
          tunnel: [w442 w451] -> w431
          tunnel: w429 -> [w440 w451]
          frame False {
            n161 = call <vilib>:"SummaryWithGlyphManager.vi"("error in"=w445, "glyph manager"=w440, "node self ref"=w444) -> ("error out"=w447:errorcluster, "glyph manager out"=w441:T9, "summary"=w446:T18[])  [unwired: 6 in]
            n162 = call <vilib>:"RefreshSubTreeWithGlyphManager.vi"("error in"=w447, "glyph manager"=w441, "node information"=w446, "tree ref in"=w443) -> ("error out"=w450:errorcluster, "glyph manager out"=w442:T9, "tree ref out"=w448:refnum<vi>)  [unwired: 5 in]
            n163 = Close Reference(reference=w448, error in (no error)=w450) -> (error out=w449:errorcluster)
          }
          frame True {
          }
        }
        n164 = Bundle By Name(cluster=w430, "glyph manager"=w431) -> (w438:T1)
      }
      frame "RemoveNode" {
        n165 = call <vilib>:"IDtoNode.vi"("error in"=w458, "ID"=w459) -> ("error out"=w457:errorcluster, "invalid Id"=w454:bool, "node ref"=w456:T2)  [unwired: 7 in]
        n166 = case shown="False" w454 {
          tunnel: w457 -> [w466 w467]
          tunnel: w456 -> [w465 _]
          tunnel: [w462 w467] -> w455
          tunnel: w453 -> [w461 _]
          frame False {
            n167 = call <vilib>:"RemoveNode.vi"("error in"=w466, "node"=w465) -> ("error out"=w463:errorcluster, "node ID"=w464:string)  [unwired: 8 in]
            n168 = call <vilib>:"ClearTreeNode.vi"("error in"=w463, "tag"=w464, "tree reference"=w461) -> ("error out"=w462:errorcluster)  [unwired: 8 in]
          }
          frame True {
          }
        }
      }
      frame "PopulateTree" {
        n169 = Unbundle By Name(w490) -> ("standard events"=w482:T3, "glyph manager"=w479:T9, "root"=w486:T2)
        n170 = String Length(string=w471) -> (length=w470:i32)
        n171 = Greater Than 0?(x=w470) -> (x > 0?=w469:bool)
        n172 = call <vilib>:"SummaryWithGlyphManager.vi"("error in"=w488, "glyph manager"=w479, "depth"=0 ("Depth"), "node self ref"=w486) -> ("error out"=w487:errorcluster, "glyph manager out"=w478:T9, "summary"=w474:T18[])  [unwired: 5 in]
        n173 = Index Array(array=w474) -> (element=w473:T18)  [unwired: 1 in]
        n174 = control-ref of="This VI"() -> (w489:refnum<vi>)
        n175 = Unbundle By Name(w473) -> ("ID"=w472:string)
        n176 = call <vilib>:"RefreshEntireTreeWithGlyphManager.vi"("calling VI in"=w489, "error in"=w487, "glyph manager"=w478, "array"=w474, "tree ref in"=w477) -> ("error out"=w483:errorcluster, "glyph manager out"=w480:T9)  [unwired: 5 in]
        n177 = control-ref of="Sub Panel"() -> (w484:refnum<vi>)
        n178 = call <vilib>:"ClearSubPanelStandardEvents.vi"("error in"=w483, "standard events"=w482, "sub panel ref in"=w484) -> ("error out"=w476:errorcluster)  [unwired: 7 in, 1 out]
        n179 = Bundle By Name(cluster=w490, "glyph manager"=w480) -> (w481:T1)
        n180 = disable-structure shown="Enabled" {
          disable-tunnel: w477 -> [w493 w497]
          disable-tunnel: w476 -> [w492 w499]
          disable-tunnel: [w491 w498] -> w475
          disable-tunnel: w472 -> [_ w496]
          disable-tunnel: w469 -> [_ w495]
          frame Disabled {
            # "#Change - Condense tree"
            n181 = invoke class="Tree (strict)" method="Open/Close.Open/Close All"(reference=w493, error in=w492, "Open"=FALSE ("Open?")) -> (error out=w491:errorcluster)  [unwired: 1 in, 3 out]
          }
          frame Enabled {
            n182 = case shown="True" w495 {
              tunnel: w499 -> [w500 w504]
              tunnel: [w500 w503] -> w498
              tunnel: w497 -> [_ w502]
              tunnel: w496 -> [_ w501]
              frame False {
              }
              frame True {
                n183 = property class="Tree (strict)"(reference=w502, error in=w504, "Val(Sgnl)"=w501) -> (error out=w503:errorcluster)  [unwired: 1 out]
              }
            }
          }
        }
        n184 = local write "Status"("" ("Status")) -> ()
      }
      frame "CleansubPanel" {
        n185 = Unbundle By Name(w509) -> ("standard events"=w505:T3)
        n186 = control-ref of="Sub Panel"() -> (w511:refnum<vi>)
        n187 = call <vilib>:"ClearSubPanelStandardEvents.vi"("error in"=w510, "standard events"=w505, "sub panel ref in"=w511) -> ("error out"=w508:errorcluster, "sub panel ref out"=w507:refnum<vi>)  [unwired: 7 in]
        n188 = Close Reference(reference=w507, error in (no error)=w508) -> (error out=w506:errorcluster)
      }
      frame "ActivateNode" {
        n189 = Unbundle By Name(w514) -> ("standard events"=w513:T3)
        n190 = call <vilib>:"IDtoNode.vi"("error in"=w519, "ID"=w520) -> ("error out"=w512:errorcluster, "invalid Id"=w518:bool, "node ref"=w517:T2)  [unwired: 7 in]
        n191 = case shown="False" w518 {
          tunnel: w517 -> [w527 _]
          tunnel: [w528 w529] -> w516
          tunnel: w512 -> [w525 w529]
          tunnel: w515 -> [w523 _]
          tunnel: w513 -> [w521 _]
          frame False {
            n192 = control-ref of="Sub Panel"() -> (w524:refnum<vi>)
            n193 = call <vilib>:"ClearSubPanelStandardEvents.vi"("error in"=w525, "standard events"=w521, "sub panel ref in"=w524) -> ("error out"=w526:errorcluster, "sub panel ref out"=w522:refnum<vi>)  [unwired: 7 in]
            n194 = call <vilib>:"LoadNodeUIStandardEvents.vi"("user event out"=w521, "error in"=w526, "sub panel ref in"=w522, "main queue"=w523, "node"=w527) -> ("error out"=w528:errorcluster)  [unwired: 6 in]
          }
          frame True {
          }
        }
      }
      frame "Move" {
        n195 = Unflatten From String(type=T14 {"node ref"=refnum, "new parent"=refnum} ("Cluster"), binary string=w540, error in (no error)=w538) -> (value=w537:T14, error out=w536:errorcluster)  [unwired: 2 in, 1 out]
        n196 = Unbundle By Name(w537) -> ("node ref"=w531:T2, "new parent"=w530:T2)
        n197 = call <vilib>:"MoveNode.vi"("error in"=w536, "new parent"=w530, "node"=w531) -> ("error out"=w534:errorcluster)  [unwired: 8 in]
        n198 = call <vilib>:"Send Local Message.vi"("message queue in"=w532, "message name"="PopulateTree", "error in"=w534) -> ("error out"=w533:errorcluster)  [unwired: 10 in, 2 out]
      }
      frame "NodeDataChange" {
        n199 = call <vilib>:"Send Local Message.vi"("message queue in"=w545, "message name"="RefreshNode", "message value"=w547, "error in"=w548) -> ("error out"=w546:errorcluster)  [unwired: 9 in, 2 out]
        n200 = Bundle By Name(cluster=w549, "unsaved changes"=TRUE) -> (w543:T1)
      }
    }
  }
  n201 = while "User Interface Event Handler" {
    tunnel: w25 -> [w558]
    tunnel: w24 -> [w554]
    tunnel: w17 -> [w553]
    tunnel: [w552] -> w13
    shift-right: [w550] -> _
    shift-left: w9 -> [w551]
    stop <- w557 stop-if-true
    n202 = event shown="[0] Timeout" {
      selector: w553 -> [_ _ _ _ _ _ _ _ _ _ _ _ _]
      dyn-events: [_ _ _ _ _ _ _ _ _ _ _ _ _] -> w552
      timeout: 1000 -> [_ _ _ _ _ _ _ _ _ _ _ _ _]
      tunnel: w558 -> [w562 w571 w596 w643 w650 w678 w707 w715 w745 w750 w761 w768 w815]
      tunnel: [_ _ _ _ _ _ TRUE _ _ _ _ _ _] -> w557
      tunnel: [w562 w571 w595 w643 w650 w676 w703 w715 w742 w750 w759 w767 w816] -> w556
      tunnel: [w561 w567 w594 _ w644 w675 w704 w711 w741 w747 w757 w765 _] -> w555
      tunnel: w554 -> [w561 w570 w593 _ w645 w677 w705 w714 w740 w749 w758 w766 _]
      tunnel: w551 -> [w560 w563 w589 w641 w646 w662 w702 w710 w739 w746 w756 w763 w813]
      tunnel: [w560 w563 w589 w641 w647 w662 w702 w710 w739 w746 w756 w763 w813] -> w550
      event Timeout {
        # "Timeout code can be added here for autosave or Lock Screen"
        n203 = event-data() -> ()  [unwired: 1 in, 1 out]
      }
      event "View": Shortcut Menu Activation? {
        n204 = event-data() -> ("CtlRef"=w577:refnum<vi>, "Coords"=w576:T19, "MenuRef"=w573:refnum<k9>)  [unwired: 1 in]
        n205 = invoke class="Tree (strict)" method="Point To Row Column"(reference=w577, error in=w570, "Point"=w576) -> (error out=w569:errorcluster, "Tag"=w575:string)  [unwired: 5 in, 6 out]
        n206 = call <vilib>:"IDtoNode.vi"("error in"=w569, "ID"=w575) -> ("error out"=w565:errorcluster, "invalid Id"=w572:bool, "node ref"=w574:T2)  [unwired: 7 in]
        n207 = case shown="False" w572 {
          tunnel: w574 -> [w582 _]
          tunnel: w573 -> [w581 _]
          tunnel: [w580 _] -> w568
          tunnel: [w579 _] -> w566
          tunnel: w565 -> [w578 w588]
          tunnel: [w578 w588] -> w564
          frame False {
            n208 = in-place {
              in-place-border: w581 -> [w585]
              in-place-border: [w583] -> w580
              n209 = in-place-dvr #8(w582) -> (w587:refnum<class "NISE_CEF_Node.lvclass">, w584:errorcluster)
              n210 = call-dynamic "ShortcutMenu.vi"("error in"=w584, "menu ref in"=w585, "node in"=w587) -> ("error out"=w583:errorcluster, "node out"=w586:refnum<class "NISE_CEF_Node.lvclass">)  [unwired: 6 in, 1 out]
              n211 = in-place-dvr #8(w586) -> (w579:errorcluster)  [unwired: 1 out]
            }
          }
          frame True {
          }
        }
        n212 = Merge Errors(w566, w568, w564) -> (w567:errorcluster)
        n213 = event-data() -> ()  [unwired: 2 in, 1 out]
      }
      event "View": Shortcut Menu Selection (User) {
        n214 = event-data() -> ("ItemPath"=w590:string, "CtlRef"=w599:refnum<vi>, "Coords"=w600:T19)  [unwired: 1 in]
        n215 = invoke class="Tree (strict)" method="Point To Row Column"(reference=w599, error in=w593, "Point"=w600) -> (error out=w592:errorcluster, "Tag"=w591:string)  [unwired: 5 in, 6 out]
        n216 = Match Pattern(string=w590, regular expression=":") -> (before substring=w598:string, after substring=w597:string)  [unwired: 1 in, 2 out]
        n217 = case shown="\"Add\"" w598 {
          selector: w598 -> [w602 _ _ _ _]
          tunnel: w597 -> [_ _ _ w626 w630]
          tunnel: w596 -> [w609 w616 w622 w628 w637]
          tunnel: w591 -> [w604 w614 w620 w625 w636]
          tunnel: [w606 w613 w619 w624 w634] -> w595
          tunnel: [w607 w612 w617 w623 w632] -> w594
          tunnel: w592 -> [w608 w611 w618 w627 w633]
          frame Default {
            n218 = Concatenate Strings(w602, ":" ("string"), w604) -> (w605:string)
            n219 = call <vilib>:"Send Local Message.vi"("message queue in"=w609, "message name"="CustomMenuAction" ("Message Name"), "message value"=w605, "error in"=w608) -> ("message queue out"=w606:T12, "error out"=w607:errorcluster)  [unwired: 9 in, 1 out]
          }
          frame "Remove" {
            n220 = call <vilib>:"Send Local Message.vi"("message queue in"=w616, "message name"="RemoveNode" ("Message Name"), "message value"=w614, "error in"=w611) -> ("message queue out"=w613:T12, "error out"=w612:errorcluster)  [unwired: 9 in, 1 out]
          }
          frame "Duplicate" {
            n221 = call <vilib>:"Send Local Message.vi"("message queue in"=w622, "message name"="Duplicate" ("Message Name"), "message value"=w620, "error in"=w618) -> ("message queue out"=w619:T12, "error out"=w617:errorcluster)  [unwired: 9 in, 1 out]
          }
          frame "Add" {
            n222 = call "Send Message to Create Child Object.vi"("Error In"=w627, "ID of Node to Add To"=w625, "node type"=w626, "Queue in"=w628) -> ("Error Out"=w623:errorcluster, "Queue Out"=w624:T12)  [unwired: 6 in]
          }
          frame "New" {
            n223 = Match Pattern(string=w630, regular expression=":") -> (after substring=w629:string)  [unwired: 1 in, 3 out]
            n224 = Bundle By Name(cluster=T13 {"node type"="", "to add to"=""} ("input cluster"), "node type"=w629, "to add to"=w636) -> (w638:T13)
            n225 = Flatten To String(anything=w638) -> (data string=w639:string)  [unwired: 3 in, 2 out]
            n226 = call <vilib>:"Send Local Message.vi"("message queue in"=w637, "message name"="AddNode" ("Message Name"), "message value"=w639, "error in"=w633) -> ("message queue out"=w634:T12, "error out"=w632:errorcluster)  [unwired: 9 in, 1 out]
          }
        }
      }
      event "VeriStand Version": Value Change {
        n227 = event-data() -> ()  [unwired: 1 in, 6 out]
        n228 = global write "Global Settings.vi" "VeriStand Version"("VeriStand Version") -> ()
      }
      event "Target Project": Value Change {
        n229 = event-data() -> ("OldVal"=w648:string)  [unwired: 1 in, 5 out]
        n230 = case shown="Default" "Target Project" {
          selector: "Target Project" -> [_ w660]
          tunnel: w648 -> [w655 _]
          tunnel: [w653 w659] -> w647
          tunnel: w646 -> [_ w659]
          tunnel: w645 -> [w652 w658]
          tunnel: [w651 w657] -> w644
          frame "Refresh..." {
            n231 = control-ref of="Target Project"() -> (w656:refnum<vi>)
            n232 = call "Initialize Target Project.vi"("error in (no error)"=w652, "ComboBox in"=w656) -> ("error out"=w654:errorcluster, "Projects"=w653:T11)  [unwired: 8 in]
            n233 = call "Set Target Project.vi"("error in (no error)"=w654, "Target Project"=w655, "Projects"=w653, "ComboBox Ref"=w656) -> ("error out"=w651:errorcluster)  [unwired: 7 in]
          }
          frame Default {
            n234 = control-ref of="Target Project"() -> (w661:refnum<vi>)
            n235 = call "Set Target Project.vi"("error in (no error)"=w658, "Target Project"=w660, "Projects"=w659, "ComboBox Ref"=w661) -> ("error out"=w657:errorcluster)  [unwired: 7 in]
          }
        }
      }
      event "View": Drop {
        n236 = event-data() -> ("CtlRef"=w681:refnum<vi>, "Coords"=w680:T19)  [unwired: 1 in]
        n237 = invoke class="Tree (strict)" method="Point To Row Column"(reference=w681, error in=w677, "Point"=w680) -> (reference out=w679:refnum<vi>, error out=w674:errorcluster, "Tag"=w671:string)  [unwired: 5 in, 5 out]
        n238 = call <vilib>:"ValidDragDrop.vi"("error in"=w674, "drag over"=w671, "Tree Ref in"=w679) -> ("Error Out"=w666:errorcluster, "Accepted"=w669:bool, "Drag"=w673:string, "Tree Ref out"=w683:refnum<vi>)  [unwired: 1 in, 4 out]
        n239 = call <vilib>:"IDtoNode.vi"("error in"=w666, "ID"=w671) -> ("error out"=w667:errorcluster, "invalid Id"=w664:bool, "node ref"=w670:T2)  [unwired: 7 in]
        n240 = call <vilib>:"IDtoNode.vi"("error in"=w667, "ID"=w673) -> ("error out"=w665:errorcluster, "invalid Id"=w663:bool, "node ref"=w672:T2)  [unwired: 7 in]
        n241 = Compound Arithmetic op=AND(w669, invert w664, invert w663) -> (w668:bool)
        n242 = case shown="True" w668 {
          tunnel: w673 -> [_ w699]
          tunnel: w683 -> [_ w701]
          tunnel: [_ TRUE] -> w682
          tunnel: w671 -> [_ w697]
          tunnel: w678 -> [w685 w696]
          tunnel: [w685 w692] -> w676
          tunnel: [w684 w691] -> w675
          tunnel: w672 -> [_ w687]
          tunnel: w670 -> [_ w686]
          tunnel: w665 -> [w684 w688]
          frame False {
          }
          frame True {
            n243 = invoke class="Tree (strict)" method="Edit Tree Items.Move Item"(reference=w701, error in=w688, "tag"=w699, "New Parent"=w697) -> (error out=w689:errorcluster)  [unwired: 3 in, 6 out]
            n244 = Bundle By Name(cluster=T14 {"node ref"=refnum, "new parent"=refnum} ("Cluster"), "new parent"=w686, "node ref"=w687) -> (w695:T14)
            n245 = Flatten To String(anything=w695, error in (no error)=w689) -> (data string=w694:string, error out=w690:errorcluster)  [unwired: 2 in, 1 out]
            n246 = call <vilib>:"Send Local Message.vi"("message queue in"=w696, "message name"="Move", "message value"=w694, "error in"=w690) -> ("message queue out"=w692:T12, "error out"=w691:errorcluster)  [unwired: 9 in, 1 out]
          }
        }
        n247 = event-data("Accepted?"=w682) -> ()  [unwired: 1 in, 1 out]
      }
      event "Exit": Value Change {
        # "Exit the application                                           >> Stop this message generator loop    Cleaning errors if the other loop stop this one"
        n248 = event-data() -> ()  [unwired: 1 in, 1 out]
        n249 = call <vilib>:"Send Local Message.vi"("message queue in"=w707, "message name"="Close", "error in"=w705) -> ("message queue out"=w703:T12, "error out"=w708:errorcluster)  [unwired: 10 in, 1 out]
        n250 = call <vilib>:"Clear Errors.vi"("error in (no error)"=w708) -> ("error out"=w704:errorcluster)  [unwired: 5 in, 1 out]
      }
      event "View": Drag Starting? {
        n251 = event-data() -> ("Data"=w721:T20, "CtlRef"=w723:refnum<vi>, "Coords"=w722:T19)  [unwired: 1 in]
        n252 = invoke class="Tree (strict)" method="Point To Row Column"(reference=w723, error in=w714, "Point"=w722) -> (error out=w713:errorcluster, "Tag"=w720:string)  [unwired: 5 in, 6 out]
        n253 = call <vilib>:"IDtoNode.vi"("error in"=w713, "ID"=w720) -> ("error out"=w712:errorcluster, "invalid Id"=w719:bool, "node ref"=w718:T2)  [unwired: 7 in]
        n254 = case shown="False" w719 {
          tunnel: w718 -> [w731 _]
          tunnel: [w728 TRUE ("Removable")] -> w716
          tunnel: w712 -> [w727 w737]
          tunnel: [w724 w737] -> w711
          frame False {
            n255 = in-place {
              in-place-border: [w734] -> w730
              in-place-border: w727 -> [w733]
              in-place-border: [w732] -> w726
              n256 = in-place-dvr #9(w731) -> (w736:refnum<class "NISE_CEF_Node.lvclass">)  [unwired: 1 out]
              n257 = call-dynamic "EditOptions.vi"("error in"=w733, "node in"=w736) -> ("error out"=w732:errorcluster, "edit options"=w734:T21, "node out"=w735:refnum<class "NISE_CEF_Node.lvclass">)  [unwired: 6 in, 1 out]
              n258 = in-place-dvr #9(w735) -> (w725:errorcluster)  [unwired: 1 out]
            }
            n259 = Unbundle By Name(w730) -> ("movable"=w729:bool)
            n260 = Merge Errors(w725, w726) -> (w724:errorcluster)
            n261 = Not(x=w729) -> (.not. x?=w728:bool)
          }
          frame True {
          }
        }
        n262 = event-data("Data"=w721, "Drag Mode"=enum32{"copy or move", "copy only", "move only"}."move only", "Discard?"=w716) -> ()  [unwired: 1 in, 1 out]
      }
      event "View": Value Change {
        n263 = event-data() -> ("NewVal"=w743:string)  [unwired: 1 in]
        n264 = call <vilib>:"Send Local Message.vi"("message queue in"=w745, "message name"="ActivateNode" ("Message Name"), "message value"=w743, "error in"=w740) -> ("message queue out"=w742:T12, "error out"=w741:errorcluster)  [unwired: 9 in, 1 out]
      }
      event "View": event type 3.0.xa000003a {
        n265 = event-data() -> ("CtlRef"=w755:refnum<vi>, "Coords"=w752:T19)  [unwired: 1 in]
        n266 = invoke class="Tree (strict)" method="Point To Row Column"(reference=w755, error in=w749, "Point"=w752) -> (reference out=w754:refnum<vi>, error out=w748:errorcluster, "Tag"=w753:string)  [unwired: 5 in, 5 out]
        n267 = call <vilib>:"ValidDragDrop.vi"("error in"=w748, "drag over"=w753, "Tree Ref in"=w754) -> ("Error Out"=w747:errorcluster, "Accepted"=w751:bool)  [unwired: 1 in, 6 out]
        n268 = event-data("Accepted?"=w751) -> ()  [unwired: 1 in, 1 out]
      }
      event Panel Close? {
        # "Intercepts the upper right close panel operation to allow a smooth shutdown as opposed to immediately killing the app."
        n269 = event-data() -> ()  [unwired: 1 in, 1 out]
        n270 = call <vilib>:"Send Local Message.vi"("message queue in"=w761, "message name"="Close?", "error in"=w758) -> ("message queue out"=w759:T12, "error out"=w757:errorcluster)  [unwired: 10 in, 1 out]
        n271 = event-data("Discard?"=TRUE) -> ()  [unwired: 1 in, 1 out]
      }
      event Menu Selection (User) {
        # "#USERCFG It is needed to add a Case for Every item on the menu"
        n272 = event-data() -> ("ItemTag"=w764:string, "ItemPath"=w769:string)  [unwired: 1 in]
        n273 = case shown="Default" w769 {
          selector: w769 -> [w773 _ _ _ _ _ _]
          tunnel: w768 -> [w778 w783 w788 w793 w798 w803 w812]
          tunnel: [w778 w779 w784 w789 w794 w799 w809] -> w767
          tunnel: w766 -> [w775 w781 w786 w791 w796 w801 w808]
          tunnel: [w774 w780 w785 w790 w795 w800 w806] -> w765
          tunnel: w764 -> [w772 _ _ _ _ _ _]
          frame Default {
            n274 = Concatenate Strings(w772, "::" ("string"), w773) -> (w771:string)
            n275 = call <vilib>:"NISE_error generator.vi"("error in"=w775, "source"="configuration tool main.vi", "append error message"=w771, "error code (0)"=538506) -> ("error out"=w774:errorcluster)  [unwired: 5 in]
          }
          frame "_File:_New" {
            n276 = call <vilib>:"Send Local Message.vi"("message queue in"=w783, "message name"="New?" ("Message Name"), "error in"=w781) -> ("message queue out"=w779:T12, "error out"=w780:errorcluster)  [unwired: 10 in, 1 out]
          }
          frame "_File:_Open" {
            n277 = call <vilib>:"Send Local Message.vi"("message queue in"=w788, "message name"="Open?" ("Message Name"), "error in"=w786) -> ("message queue out"=w784:T12, "error out"=w785:errorcluster)  [unwired: 10 in, 1 out]
          }
          frame "_File:_Save" {
            n278 = call <vilib>:"Send Local Message.vi"("message queue in"=w793, "message name"="Save" ("Message Name"), "error in"=w791) -> ("message queue out"=w789:T12, "error out"=w790:errorcluster)  [unwired: 10 in, 1 out]
          }
          frame "_File:Save As..." {
            n279 = call <vilib>:"Send Local Message.vi"("message queue in"=w798, "message name"="SaveAs" ("Message Name"), "error in"=w796) -> ("message queue out"=w794:T12, "error out"=w795:errorcluster)  [unwired: 10 in, 1 out]
          }
          frame "_File:_Exit" {
            n280 = call <vilib>:"Send Local Message.vi"("message queue in"=w803, "message name"="Close?" ("Message Name"), "error in"=w801) -> ("message queue out"=w799:T12, "error out"=w800:errorcluster)  [unwired: 10 in, 1 out]
          }
          frame "_Tools:Multiple Parameter Editor" {
            n281 = call <vilib>:"Send Local Message.vi"("message queue in"=w812, "message name"="CleansubPanel", "error in"=w808) -> ("message queue out"=w811:T12, "error out"=w807:errorcluster)  [unwired: 10 in, 1 out]
            n282 = call <vilib>:"Send Local Message.vi"("message queue in"=w811, "message name"="Custom View" ("Message Name"), "message value"="Multiple Variable Editor" ("Message Name"), "error in"=w807) -> ("message queue out"=w809:T12, "error out"=w806:errorcluster)  [unwired: 9 in, 1 out]
          }
        }
      }
      event User Event {
        n283 = event-data() -> ("node ref"=w814:T2)  [unwired: 1 in]
        n284 = call <vilib>:"NodetoID.vi"("node ref"=w814) -> ("ID"=w817:string)  [unwired: 9 in, 1 out]
        n285 = call <vilib>:"Send Local Message.vi"("message queue in"=w815, "message name"="NodeDataChange", "message value"=w817) -> ("message queue out"=w816:T12)  [unwired: 10 in, 2 out]
      }
    }
    n286 = call "Error.vi"("error in (no error)"=w555, "message queue in"=w556) -> ()  [unwired: 9 in, 1 out]
  }
  n287 = Unregister For Events(event registration refnum=w13) -> (error out=w14:errorcluster)  [unwired: 1 in]
  n288 = Merge Errors(w14, w19) -> (w15:errorcluster)
  n289 = call <vilib>:"DestroyStandardEvents.vi"("error in"=w15, "standard events"=w18) -> ("error out"=w4:errorcluster)  [unwired: 9 in]
  n290 = invoke class="VI" method="Save.Instrument"(error in=w4) -> (reference out=w3:refnum<vi>, error out=w2:errorcluster)  [unwired: 5 in, 4 out]
  n291 = disable-structure shown="Disabled" {
    disable-tunnel: w3 -> [w820 _]
    disable-tunnel: w2 -> [w819 _]
    frame Disabled {
      n292 = invoke class="VI" method="FP.Close"(reference=w820, error in=w819) -> ()  [unwired: 1 in, 3 out]
    }
    frame Enabled {
    }
  }
  "Status" <- "No configuration loaded" ("Status")
